vi "Parameters.vi"(8 "error in (no error)":errorcluster, 11 "Template Test Case In":refnum<class "Generate VI Names.lvclass">) -> (0 "error out":errorcluster, 2 "Parameters":T1(array[cluster]))   [LabVIEW 2026, in "Generate VI Names.lvclass"]
doc: "This VI defines the parameters used for execution. When LUnit runs the test case, it will run it once for every parameter in the array and collect the results.\n\nDuring test execution, the parameters are available in the class wire within the test VI."
uses:
  Generate VI Names.lvclass
  <vilib>/Astemes/LUnit Parameterized/Parameterized Test Case/Parameterized Test Case.lvclass
  Parameters.ctl
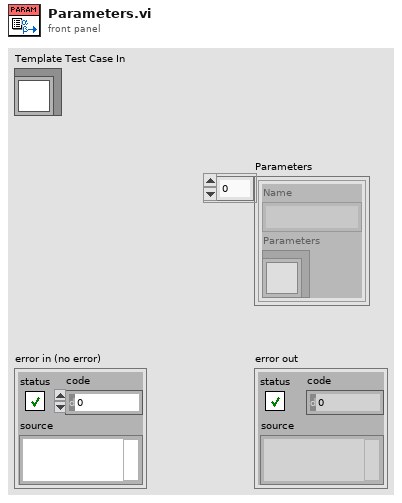
[diagram p1: front panel]
types:
  T1 = cluster{"Name":string, "Parameters":refnum<class "Parameterized Test Case.lvclass">}[]
  T2 = typedef "Generate VI Names.lvclass/Parameters.ctl" = cluster{"Python Function":string, "VI Name":string}
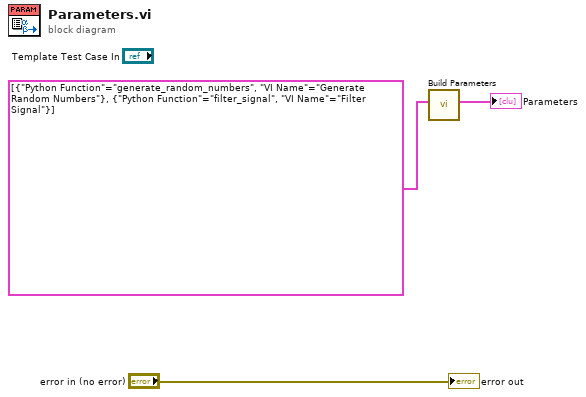
[diagram p0: block diagram]
diagram:
  n1 = call "Build Parameters.vi"("Parameters"=T2[] [{"Python Function"="generate_random_numbers", "VI Name"="Generate Random Numbers"}, {"Python Function"="filter_signal", "VI Name"="Filter Signal"}] ("Parameters 2")) -> ("Scenarios"=→"Parameters":T1)  [unwired: 10 in]
  "error out" <- "error in (no error)"
